vi "Controlleur Edwards_pompe_turbo_moleculaire_Lecture_type_de_pompe.vi"() -> ()   [LabVIEW 2022 SP3]
panel:
  in  "Énum":enum16{""}(ring)
  out "Données 1D":string[](array[string])
  out "Données Edwards":string[][](array[string])
  out "Sélection":bool[][](array[boolean])
  out "Voies":i8[][](array[numeric]) min=1 max=6 step=1
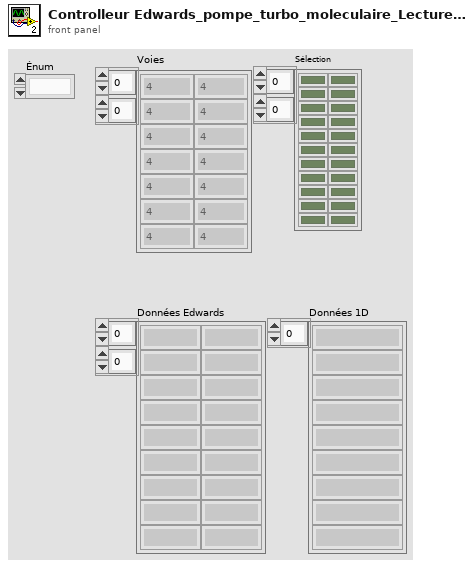
[diagram p1: front panel]
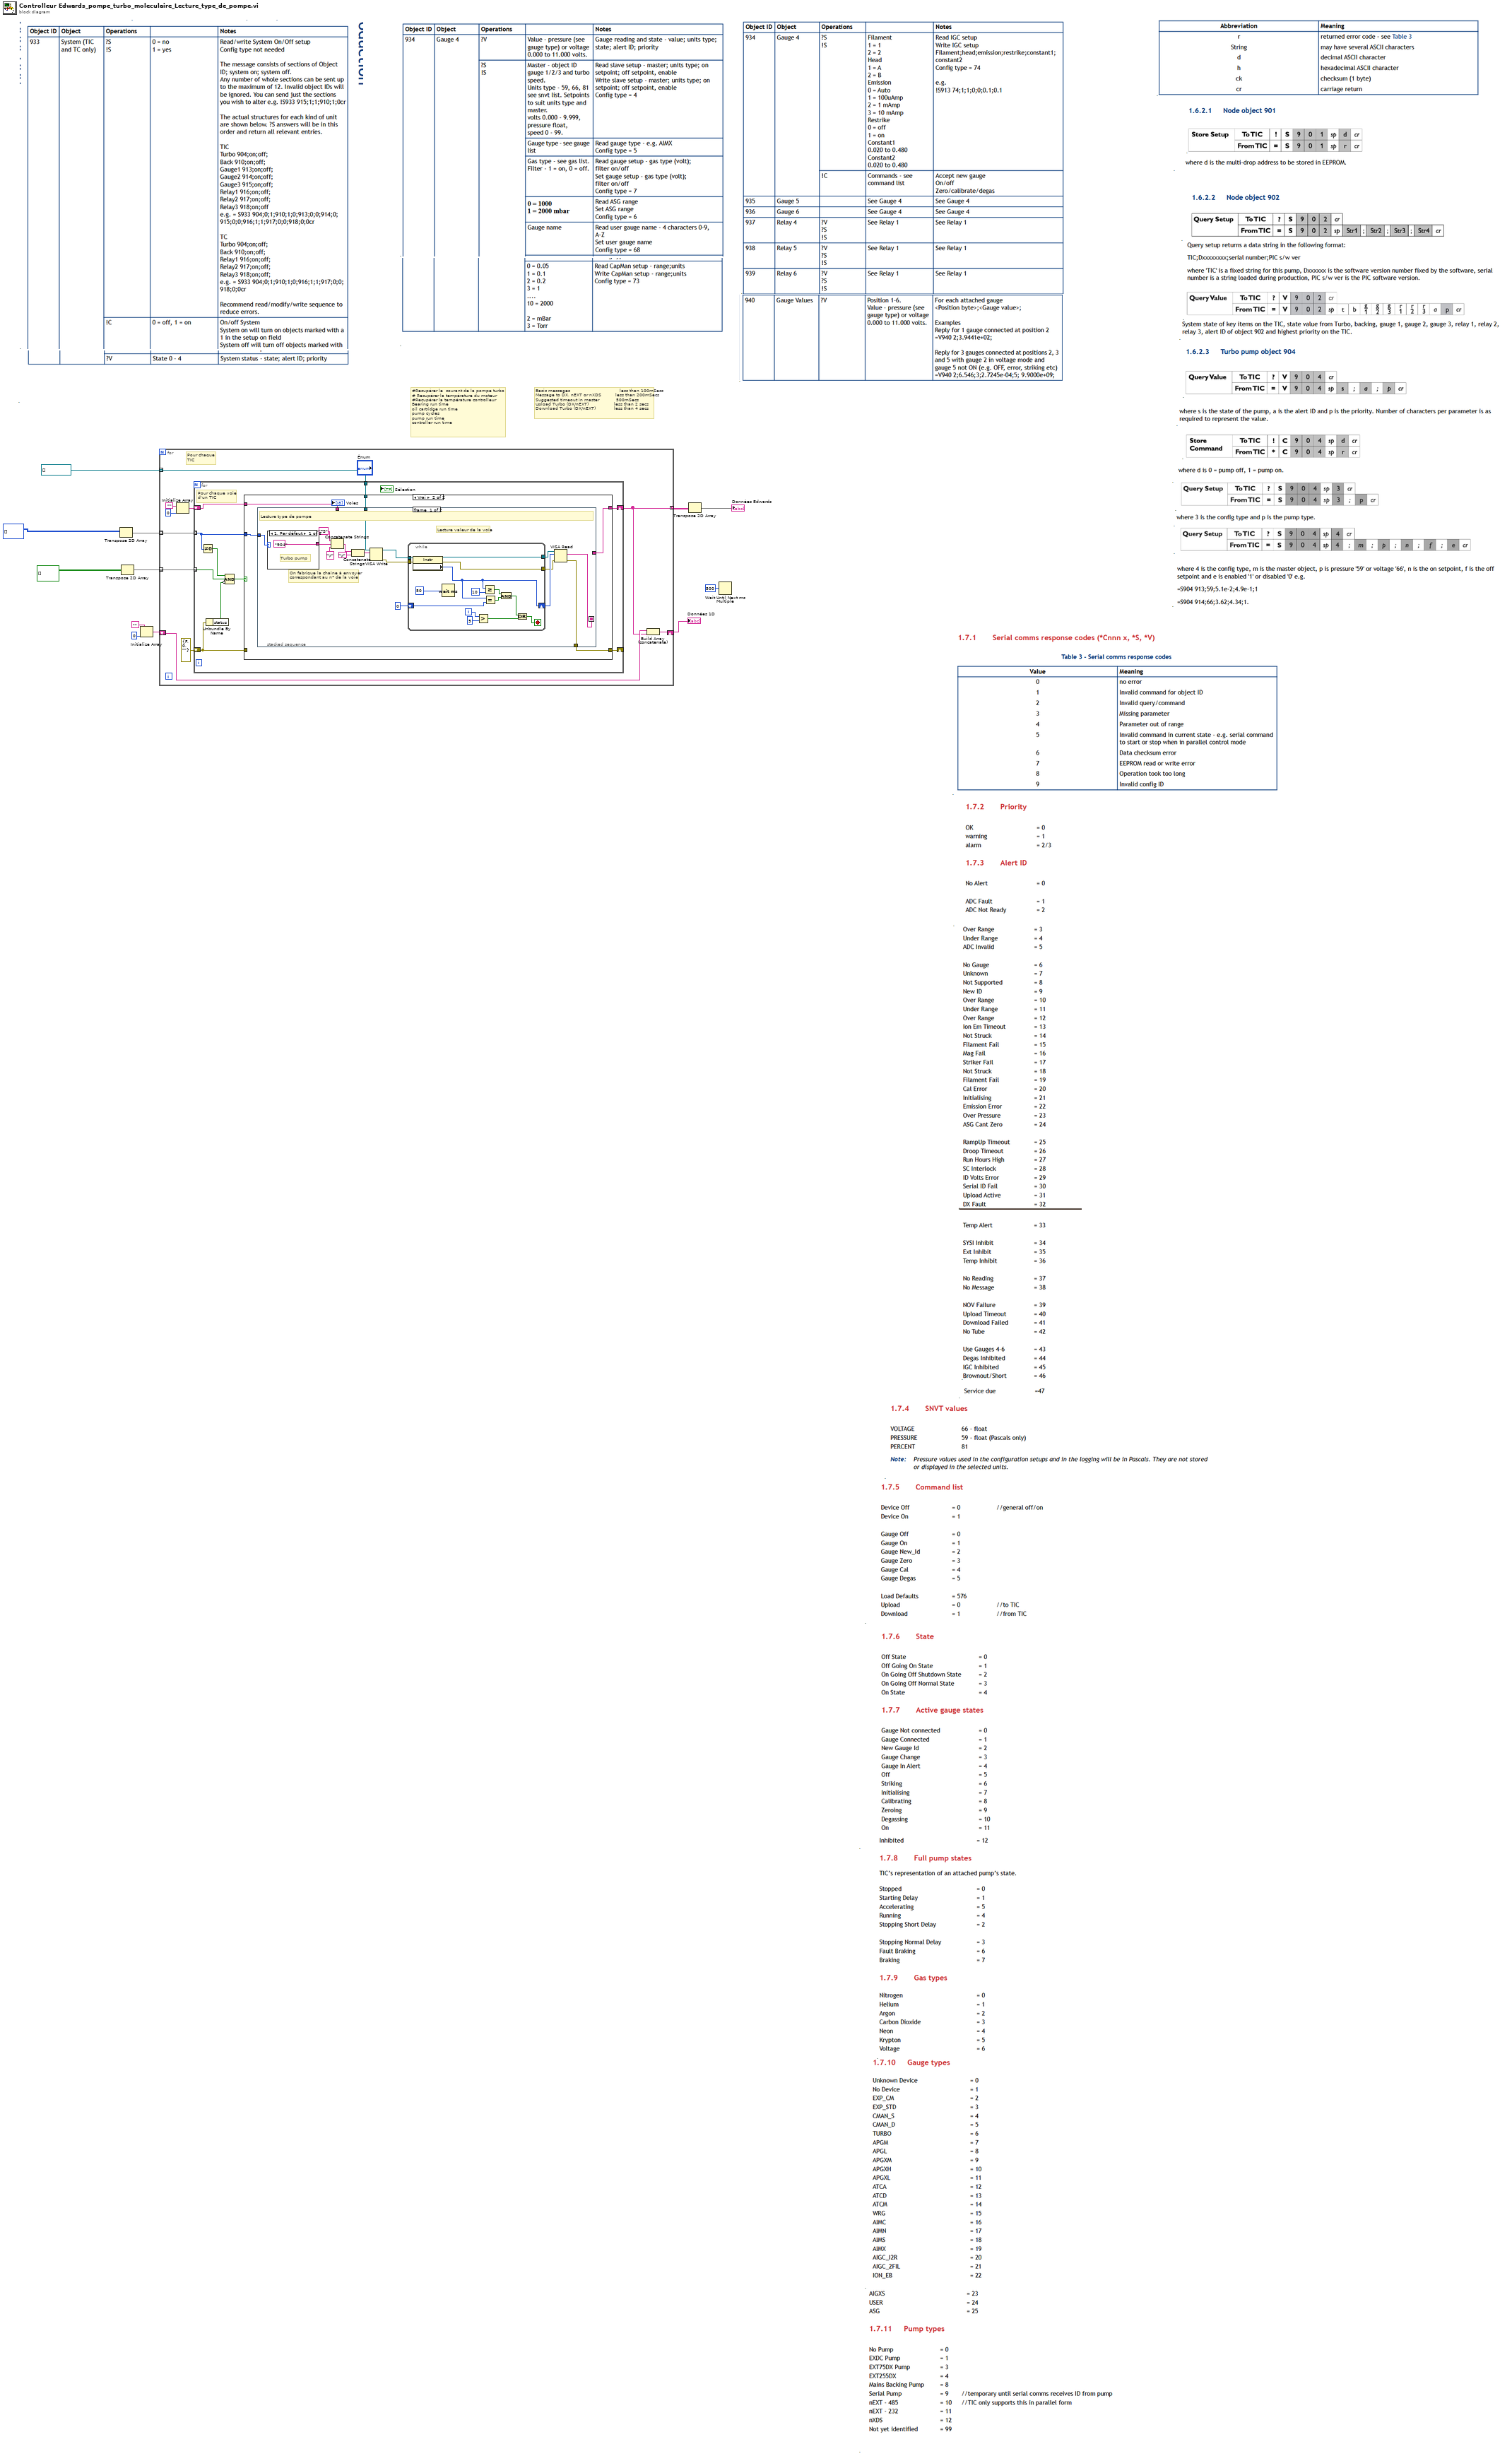
[diagram p0: block diagram]
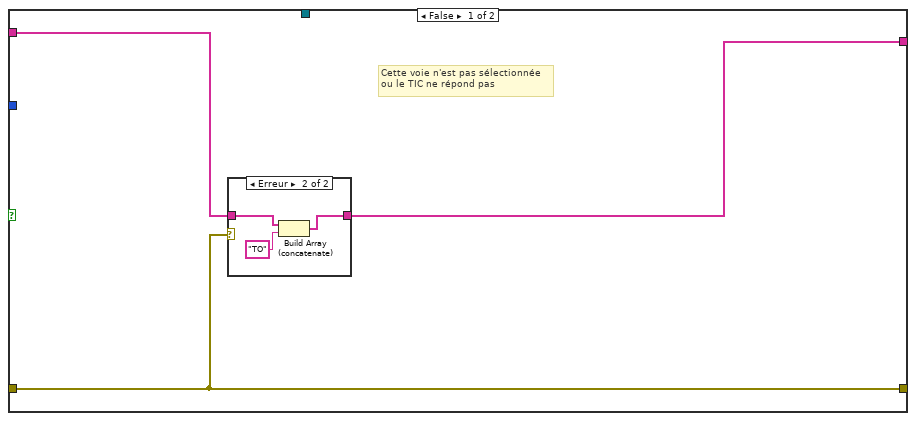
[diagram p2: hidden frame]
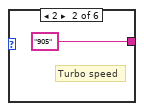
[diagram p4: hidden frame]
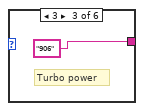
[diagram p5: hidden frame]
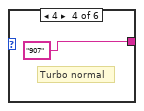
[diagram p6: hidden frame]
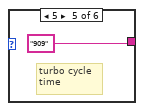
[diagram p7: hidden frame]
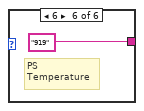
[diagram p8: hidden frame]
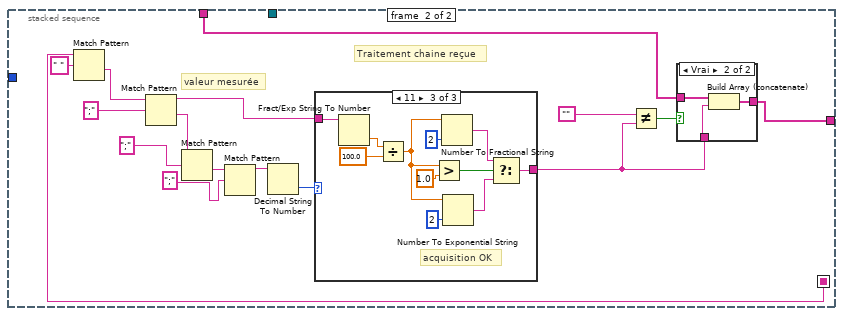
[diagram p9: hidden frame]
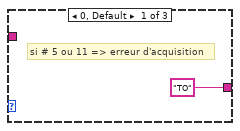
[diagram p11: hidden frame]
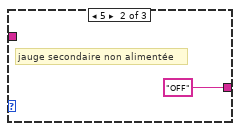
[diagram p12: hidden frame]
diagram:
  # "Basic messages                                   less than 100mSecs\nMessage to DX, nEXT or nXDS          less than 200mSecs\nSuggested timeout in master            500mSecs\nUpload Turbo (DX/nEXT)                  less than 2 secs\nDownload Turbo (DX/nEXT)             less than 4 secs"
  # "#Recupérer le  courant de la pompe turbo\n# Recupérer la température du moteur \n#Recupérer la température controlleur \nBearing run time\noil cartridge run time \npump cycles \npump run time \ncontroller run time"
  n1 = Transpose 2D Array(2D array=i8[][] [] ("Voies")) -> (transposed array=w6:i8[][])
  n2 = Transpose 2D Array(2D array=bool[][] [] ("Sélection")) -> (transposed array=w5:bool[][])
  n3 = Initialize Array("", 0 ("taille de la dimension")) -> (w9:string[])
  n4 = for {
    tunnel: w6 -> [w22] mode=indexing
    tunnel: [w15] -> w12 mode=indexing
    tunnel: w5 -> [w18] mode=indexing
    tunnel: refnum<visa-resource-name>[] [] ("Port RS232 Edwards") -> [w14] mode=indexing
    shift-right: [w16] -> w4
    shift-left: w9 -> [w17]
    # "Pour chaque\nTIC"
    n5 = Initialize Array("", 0 ("taille de la dimension")) -> (w19:string[])
    n6 = for {
      tunnel: w22 -> [w29] mode=indexing
      tunnel: w14 -> [w32]
      shift-right: [w31] -> w15
      shift-left: w19 -> [w30]
      tunnel: w18 -> [w26] mode=indexing
      shift-right: [w28] -> _
      shift-left: errorcluster {"status"=FALSE, "code"=0, "source"=""} ("error out") -> [w24]
      # "Pour chaque voie\nd'un TIC"
      n7 = Not Equal To 0?(x=w29) -> (x != 0?=w27:bool)
      n8 = Unbundle By Name(w24) -> ("status"=w23:bool)
      n9 = Compound Arithmetic op=AND ("Opérateur arithmétique")(w27, w26, invert w23) -> (w25:bool)
      n10 = case shown="Vrai" w25 {
        tunnel: w29 -> [_ w43]
        tunnel: w32 -> [_ w44]
        tunnel: [w33 w41] -> w31
        tunnel: w30 -> [w34 w42]
        tunnel: [w35 w40] -> w28
        tunnel: w24 -> [w35 _]
        frame False {
          # "Cette voie n'est pas sélectionnée\nou le TIC ne répond pas"
          n11 = case shown="Erreur" w35 {
            tunnel: w34 -> [w36 w39]
            tunnel: [w36 w38] -> w33
            frame No Error {
            }
            frame Error {
              n12 = Build Array (concatenate)(w39, "TO") -> (w38:string[])
            }
          }
        }
        frame True {
          n13 = stacked-sequence {
            seq-local: [w47 _] -> [_ w87]
            tunnel: w44 -> [w51 _]
            tunnel: w43 -> [w48 _]
            tunnel: w42 -> [_ w84]
            tunnel: [_ w82] -> w41
            tunnel: [w45 _] -> w40
            frame #0 {
              # "Lecture valeur de la voie"
              # "On fabrique la chaine à envoyer\ncorrespondant au n° de la voie"
              # "Lecture type de pompe"
              n14 = case shown="1, Par défaut" w48 {
                tunnel: ["904" "905" "906" "907" "909" "919"] -> w49
                frame 1, Default {
                  # "Turbo pump"
                }
                frame 2 {
                  # "Turbo speed"
                }
                frame 3 {
                  # "Turbo power"
                }
                frame 4 {
                  # "Turbo normal"
                }
                frame 5 {
                  # "turbo cycle \ntime"
                }
                frame 6 {
                  # "PS \nTemperature"
                }
              }
              n15 = Concatenate Strings("?S", w49, "\r") -> (w53:string)
              n16 = Concatenate Strings(w53, "\r") -> (w50:string)
              n17 = VISA Write(VISA resource name=w51, write buffer=w50) -> (VISA resource name out=w56:refnum<visa-resource-name>, error out=w46:errorcluster)  [unwired: 1 in, 1 out]
              n18 = while {
                tunnel: w56 -> [w81]
                tunnel: [w74] -> w60
                shift-right: [w73] -> w59
                shift-left: 0 -> [w72]
                tunnel: w46 -> [w68]
                tunnel: [w67] -> w52
                i -> [w79]
                stop <- w80 stop-if-true
                n19 = property class="Instr"(reference=w81, error in=w68) -> (reference out=w74:refnum<visa-resource-name>, error out=w67:errorcluster, "Serial Settings:Number of Bytes at Serial Port"=w73:u32)
                n20 = Wait (ms)(milliseconds to wait=u32 50 ("attente (ms)")) -> ()  [unwired: 1 out]
                n21 = Greater?(x=w79, y=5) -> (0:w77:bool)
                n22 = Greater Or Equal?(x=w73, y=u32 10) -> (x >= y?=w70:bool)
                n23 = Equal?(x=w73, y=w72) -> (x = y?=w71:bool)
                n24 = And(x=w70, y=w71) -> (x .and. y?=w69:bool)
                n25 = Or(x=w69, y=w77) -> (x .or. y?=w80:bool)
              }
              n26 = VISA Read(VISA resource name=w60, byte count=w59, error in (no error)=w52) -> (read buffer=w47:string, error out=w45:errorcluster)  [unwired: 2 out]
            }
            frame #1 {
              # "valeur mesurée"
              # "Traitement chaine reçue"
              n27 = Match Pattern(string=w87, regular expression=" " ("expression régulière")) -> (after substring=w89:string)  [unwired: 1 in, 3 out]
              n28 = Match Pattern(string=w89, regular expression=";" ("expression régulière")) -> (before substring=w93:string, after substring=w92:string)  [unwired: 1 in, 2 out]
              n29 = Match Pattern(string=w92, regular expression=";" ("expression régulière")) -> (after substring=w94:string)  [unwired: 1 in, 3 out]
              n30 = Match Pattern(string=w94, regular expression=";" ("expression régulière")) -> (before substring=w96:string)  [unwired: 1 in, 3 out]
              n31 = Decimal String To Number(string=w96) -> (number=w97:i32)  [unwired: 2 in, 1 out]
              n32 = case shown="11" w97 {
                tunnel: w93 -> [_ _ w114]
                tunnel: ["TO" "OFF" w108] -> w83
                frame 0, Default {
                  # "si # 5 ou 11 => erreur d'acquisition"
                }
                frame 5 {
                  # "jauge secondaire non alimentée"
                }
                frame 11 {
                  # "acquisition OK"
                  n33 = Fract/Exp String To Number(string=w114) -> (number=w113:dbl)  [unwired: 3 in, 1 out]
                  n34 = Divide(x=w113, y=100.0) -> (x/y=w105:dbl)
                  n35 = Greater?(x=w105, y=1.0) -> (0:w106:bool)
                  n36 = Number To Fractional String(number=w105, precision (6)=i16 2 ("précision (6)")) -> (F-format string=w109:string)  [unwired: 2 in]
                  n37 = Number To Exponential String(number=w105, precision (6)=i16 2 ("précision (6)")) -> (E-format string=w104:string)  [unwired: 2 in]
                  n38 = Select(t=w109, s=w106, f=w104) -> (s? t:f=w108:string)
                }
              }
              n39 = Not Equal?(x="", y=w83) -> (x != y?=w86:bool)
              n40 = case shown="Vrai" w86 {
                tunnel: w84 -> [w98 w101]
                tunnel: w83 -> [_ w100]
                tunnel: [w98 w99] -> w82
                frame False {
                }
                frame True {
                  n41 = Build Array (concatenate)(w101, w100) -> (w99:string[])
                }
              }
            }
          }
        }
      }
    }
    n42 = Build Array (concatenate)(w17, w15) -> (w16:string[])
  }
  "Données 1D" <- w4
  n43 = Transpose 2D Array(2D array=w12) -> (transposed array=→"Données Edwards":string[][])
  n44 = Wait Until Next ms Multiple(millisecond multiple=u32 500 ("n millisecondes")) -> ()  [unwired: 1 out]
